vi "VIH Project - Container - HHP Generation.vi"(7 "cmd (get)":enum16{"get", "set"}(ring), 11 "HHP_Generation in":T1={"HHP_Template"=enum."default", "HHP_Template_CustomPath"=path "", "HHP_Target"=enum."default", "HHP_Target_CustomPath"=path "", "HHP_CreateTOC"=TRUE, "HHP_CreateIDX"=TRUE, "HHP_DefaultTopic"=enum."auto", "HHP_DefaultTopic_CustomPath"=path "", "CHM_Filename"=path "", "HHP_AutoBuild"=FALSE, "CHM_AutoBuild"=FALSE}) -> (3 "HHP_Generation out":T1={"HHP_Template"=enum."default", "HHP_Template_CustomPath"=path "", "HHP_Target"=enum."default", "HHP_Target_CustomPath"=path "", "HHP_CreateTOC"=TRUE, "HHP_CreateIDX"=TRUE, "HHP_DefaultTopic"=enum."auto", "HHP_DefaultTopic_CustomPath"=path "", "CHM_Filename"=path "", "HHP_AutoBuild"=FALSE, "CHM_AutoBuild"=FALSE})   [LabVIEW 2014]
doc: "::: VI Helpeks :::\nCopyright (c) 2000-2026 Konstantin Shifershteyn. All rights reserved."
uses:
  _VIH CHM Project.llb/VIH - CHM Project - HHP Generation Params Cluster.ctl
panel:
  # "VI Helpeks\nCopyright (c) 2012-2026 Konstantin Shifershteyn"
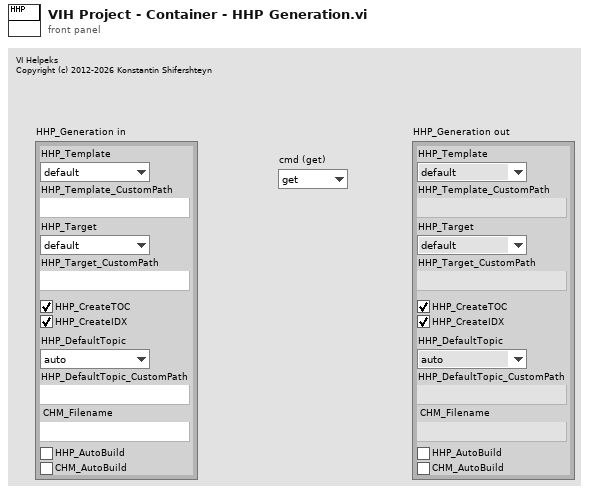
[diagram p1: front panel]
types:
  T1 = typedef "VIH - CHM Project - HHP Generation Params Cluster.ctl" = cluster{"HHP_Template":enum16{"default", "custom"}, "HHP_Template_CustomPath":path, "HHP_Target":enum16{"default", "custom"}, "HHP_Target_CustomPath":path, "HHP_CreateTOC":bool, "HHP_CreateIDX":bool, "HHP_DefaultTopic":enum16{"auto", "custom"}, "HHP_DefaultTopic_CustomPath":path, "CHM_Filename":path, "HHP_AutoBuild":bool, "CHM_AutoBuild":bool}
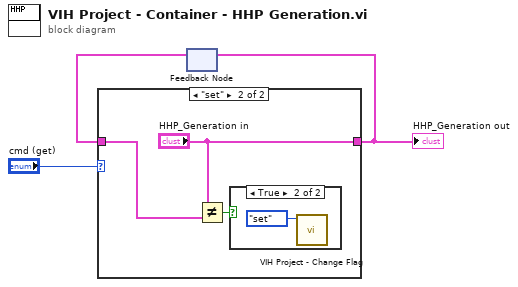
[diagram p0: block diagram]
diagram:
  n1 = feedback #1() -> (w1:T1)  [unwired: 1 in]
  n2 = case shown="\"set\"" "cmd (get)" {
    tunnel: [w4 "HHP_Generation in"] -> w2
    tunnel: w1 -> [w4 w6]
    frame "get" {
    }
    frame "set" {
      n3 = Not Equal?(x="HHP_Generation in", y=w6) -> (x != y?=w5:bool)
      n4 = case shown="True" w5 {
        frame False {
        }
        frame True {
          n5 = call "VIH Project - Change Flag.vi"("cmd (get)"=enum16{"get", "set", "reset"}."set") -> ()  [unwired: 9 in, 2 out]
        }
      }
    }
  }
  "HHP_Generation out" <- w2
  n6 = feedback-in #1(w2) -> ()
